vi "Add State.vi"(8 "error in":errorcluster, 10 "State":string, 11 "History in":refnum<class "History.lvclass">) -> (0 "error out":errorcluster, 3 "History out":refnum<class "History.lvclass">)   [LabVIEW 2020, in "lv_icon.lvlib" / "History.lvlib" / "History.lvclass"]
doc: "Adds a state to the undo stack.\n\nThis process clears the available redo states."
uses:
  History.lvclass
  History.lvclass/History.ctl
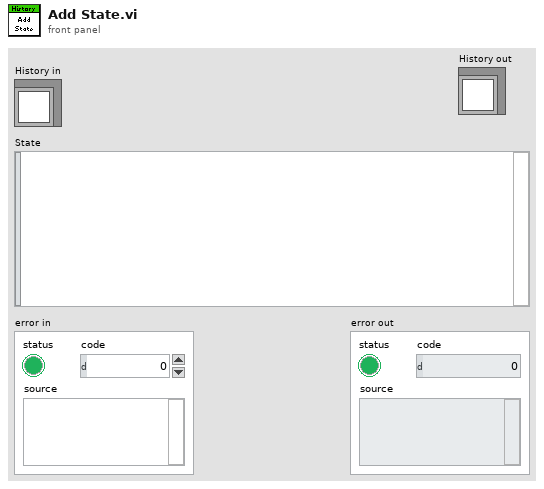
[diagram p1: front panel]
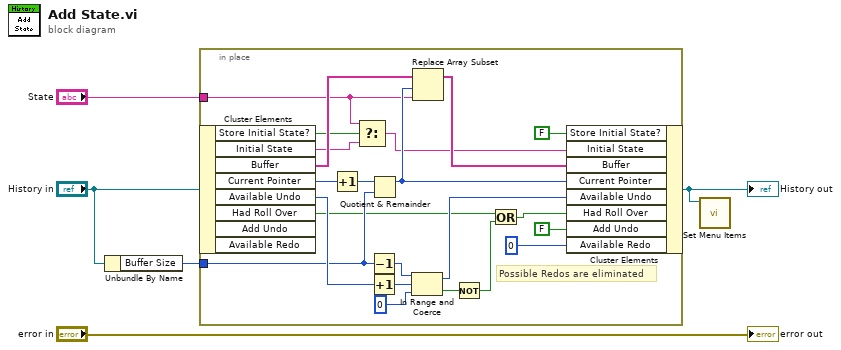
[diagram p0: block diagram]
diagram:
  n1 = Unbundle By Name("History in") -> ("Buffer Size"=w3:i32)
  n2 = in-place {
    in-place-border: w3 -> [w19]
    in-place-border: "State" -> [w8]
    # "Possible Redos are eliminated"
    n3 = in-place-cluster #1("History in") -> ("Store Initial State?"=w10:bool, "Initial State"=w7:string, "Buffer"=w18:string[], "Current Pointer"=w25:i32, "Available Undo"=w27:i32, "Had Roll Over"=w14:bool)  [unwired: 2 out]
    n4 = Increment(x=w25) -> (x+1=w26:i32)
    n5 = Select(t=w8, s=w10, f=w7) -> (s? t:f=w9:string)
    n6 = Decrement(x=w19) -> (x-1=w20:i32)
    n7 = Increment(x=w27) -> (x+1=w23:i32)
    n8 = Quotient & Remainder(x=w26, y=w19) -> (x-y*floor(x/y)=w16:i32)  [unwired: 1 out]
    n9 = In Range and Coerce(upper limit=w20, x=w23, lower limit=0) -> (coerced(x)=w15:i32, In Range?=w22:bool)
    n10 = Replace Array Subset(array=w18, new element=w8, index=w16) -> (w17:string[])
    n11 = Not(x=w22) -> (.not. x?=w21:bool)
    n12 = Or(x=w14, y=w21) -> (x .or. y?=w13:bool)
    n13 = in-place-cluster #1("Store Initial State?"=FALSE, "Initial State"=w9, "Buffer"=w17, "Current Pointer"=w16, "Available Undo"=w15, "Had Roll Over"=w13, "Add Undo"=FALSE, "Available Redo"=0) -> (w1:refnum<class "History.lvclass">)
  }
  "History out" <- w1
  n14 = call "Set Menu Items.vi"("History"=w1) -> ()  [unwired: 11 in]
  "error out" <- "error in"
